vi "Build Parameters.vi"() -> (2 "Scenarios":T1(array[cluster]))   [LabVIEW 2020]
doc: "This helper function simplifies the syntax of creating parameters."
uses:
  API Pass Output.lvclass
  Parameters.ctl
  C:/Program Files (x86)/National Instruments/LabVIEW 2020/vi.lib/Astemes/LUnit/Test Case.lvclass
  C:/Program Files (x86)/National Instruments/LabVIEW 2020/vi.lib/Astemes/LUnit/LUnit Runnable.lvclass
  C:/git/astemes-lunit/tests/API Pass Output/API Pass Output.lvclass
  <vilib>/Astemes/LUnit Parameterized/Parameterized Test Case/Parameterized Test Case.lvclass
  C:/Program Files (x86)/National Instruments/LabVIEW 2020/vi.lib/Astemes/LUnit Parameterized/Parameterized Test Case/Parameterized Test Case.lvclass
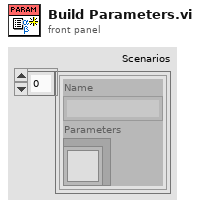
[diagram p1: front panel]
types:
  T1 = cluster{"Name":string, "Parameters":refnum<class "Parameterized Test Case.lvclass">}[]
  T2 = typedef "API Pass Output.lvclass/Parameters.ctl" = cluster{"Path":path, "Pass?":bool}
  T3 = cluster{"Scenario":string, "Parameters":refnum<class "API Pass Output.lvclass">}
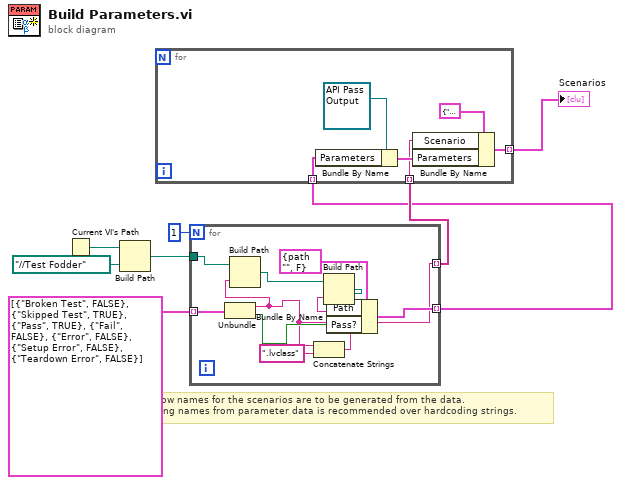
[diagram p0: block diagram]
diagram:
  # "Modify how names for the scenarios are to be generated from the data.\nGenerating names from parameter data is recommended over hardcoding strings."
  n1 = Current VI's Path() -> (path=w7:path)
  n2 = Build Path(base path=w7, name or relative path=path "../../Test Fodder") -> (appended path=w5:path)
  n3 = for {
    N: 1 -> [_]
    tunnel: w5 -> [w13]
    tunnel: cluster{string, bool}[] [{"Broken Test", FALSE}, {"Skipped Test", TRUE}, {"Pass", TRUE}, {"Fail", FALSE}, {"Error", FALSE}, {"Setup Error", FALSE}, {"Teardown Error", FALSE}] -> [w18] mode=indexing
    tunnel: [w12] -> w3 mode=indexing
    tunnel: [w16] -> w2 mode=indexing
    n4 = Unbundle(w18) -> (w12:string, w15:bool)
    n5 = Build Path(base path=w13, name or relative path=w12) -> (appended path=w11:path)
    n6 = Concatenate Strings(w12, ".lvclass" ("string")) -> (w10:string)
    n7 = Build Path(base path=w11, name or relative path=w10) -> (appended path=w9:path)
    n8 = Bundle By Name(cluster=T2 {"Path"=path "", "Pass?"=FALSE} ("Parameters"), "Path"=w9, "Pass?"=w15) -> (w16:T2)
  }
  n9 = for {
    tunnel: [w22] -> w8 mode=indexing
    tunnel: w3 -> [w20] mode=indexing
    tunnel: w2 -> [w19] mode=indexing
    n10 = Bundle By Name(cluster=refnum<class "API Pass Output.lvclass"> refnum ("Parameters"), "Parameters"=w19) -> (w23:cluster{})
    n11 = Bundle By Name(cluster=T3 {"Scenario"="", "Parameters"=refnum}, "Scenario"=w20, "Parameters"=w23) -> (w22:T3)
  }
  "Scenarios" <- w8
